vi "Test Assert Greater Or Equal.vi"(8 "error in (no error)":errorcluster) -> (0 "error out":errorcluster)   [LabVIEW 2020]
uses:
  classes/Assert/Assert.lvclass
  classes/Test/Test.lvclass
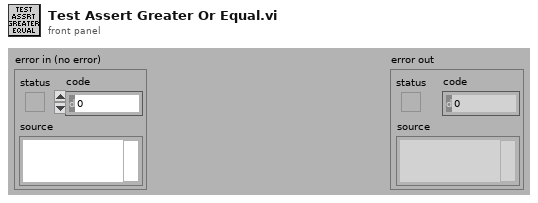
[diagram p1: front panel]
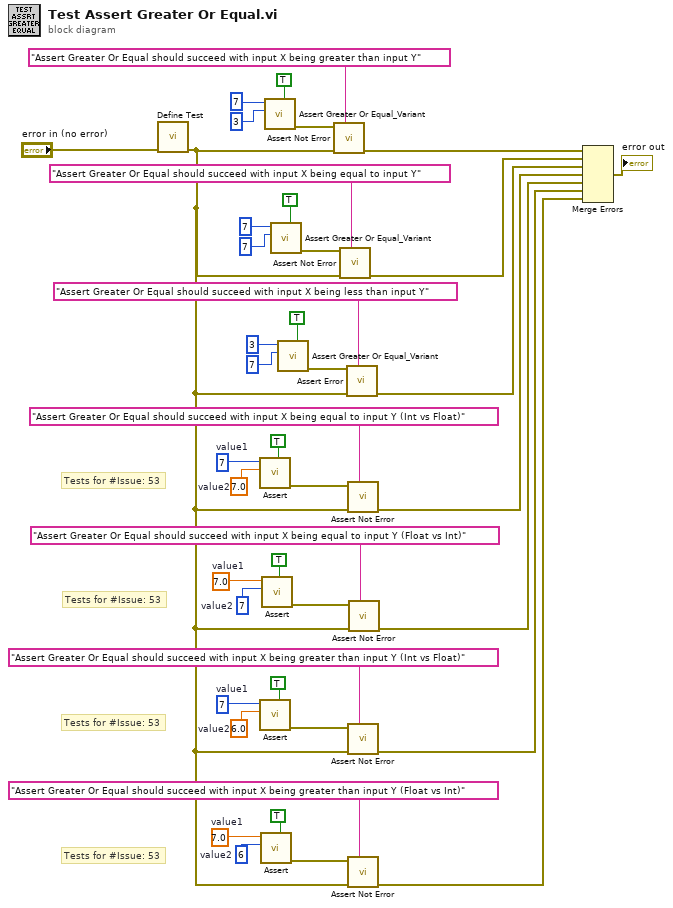
[diagram p0: block diagram]
diagram:
  w14 = 6  # value2
  w15 = 7.0  # value1
  w5 = 7  # value2
  w6 = 7.0  # value1
  w10 = 6.0  # value2
  w11 = 7  # value1
  w2 = 7.0  # value2
  w3 = 7  # value1
  # "Tests for #Issue: 53"
  # "Tests for #Issue: 53"
  # "Tests for #Issue: 53"
  # "Tests for #Issue: 53"
  n1 = call "Define Test.vi"("error in (no error)"="error in (no error)") -> ("error out"=w18:errorcluster)  [unwired: 9 in, 1 out]
  n2 = call-poly "Assert.vi"("Assert Only? (F)"=TRUE, "Y"=w2, "X"=w3) -> ("error out"=w1:errorcluster)  [unwired: 7 in, 1 out]
  n3 = call-poly "Assert.vi"("Assert Only? (F)"=TRUE, "Y"=w10, "X"=w11) -> ("error out"=w12:errorcluster)  [unwired: 7 in, 1 out]
  n4 = call-poly "Assert.vi"("Assert Only? (F)"=TRUE, "Y"=w14, "X"=w15) -> ("error out"=w13:errorcluster)  [unwired: 7 in, 1 out]
  n5 = call-poly "Assert.vi"("Assert Only? (F)"=TRUE, "Y"=w5, "X"=w6) -> ("error out"=w7:errorcluster)  [unwired: 7 in, 1 out]
  n6 = call "Assert Greater Or Equal_Variant.vi"("Assert Only? (F)"=TRUE, "Y"=3, "X"=7) -> ("error out"=w45:errorcluster)  [unwired: 7 in, 1 out]
  n7 = call "Assert Greater Or Equal_Variant.vi"("Assert Only? (F)"=TRUE, "Y"=7, "X"=7) -> ("error out"=w43:errorcluster)  [unwired: 7 in, 1 out]
  n8 = call "Assert Greater Or Equal_Variant.vi"("Assert Only? (F)"=TRUE, "Y"=7, "X"=3) -> ("error out"=w31:errorcluster)  [unwired: 7 in, 1 out]
  n9 = call "Assert Not Error.vi"("Label"="Assert Greater Or Equal should succeed with input X being greater than input Y", "error in (no error)"=w18, "Not Error?"=w45) -> ("error out"=w37:errorcluster)  [unwired: 7 in, 1 out]
  n10 = call "Assert Not Error.vi"("Label"="Assert Greater Or Equal should succeed with input X being equal to input Y", "error in (no error)"=w18, "Not Error?"=w43) -> ("error out"=w38:errorcluster)  [unwired: 7 in, 1 out]
  n11 = call "Assert Error.vi"("Label"="Assert Greater Or Equal should succeed with input X being less than input Y", "error in (no error)"=w18, "Error?"=w31) -> ("error out"=w26:errorcluster)  [unwired: 7 in, 1 out]
  n12 = call "Assert Not Error.vi"("Label"="Assert Greater Or Equal should succeed with input X being equal to input Y (Int vs Float)", "error in (no error)"=w18, "Not Error?"=w1) -> ("error out"=w25:errorcluster)  [unwired: 7 in, 1 out]
  n13 = call "Assert Not Error.vi"("Label"="Assert Greater Or Equal should succeed with input X being greater than input Y (Int vs Float)", "error in (no error)"=w18, "Not Error?"=w12) -> ("error out"=w22:errorcluster)  [unwired: 7 in, 1 out]
  n14 = call "Assert Not Error.vi"("Label"="Assert Greater Or Equal should succeed with input X being greater than input Y (Float vs Int)", "error in (no error)"=w18, "Not Error?"=w13) -> ("error out"=w17:errorcluster)  [unwired: 7 in, 1 out]
  n15 = call "Assert Not Error.vi"("Label"="Assert Greater Or Equal should succeed with input X being equal to input Y (Float vs Int)", "error in (no error)"=w18, "Not Error?"=w7) -> ("error out"=w20:errorcluster)  [unwired: 7 in, 1 out]
  n16 = Merge Errors(w37, w38, w26, w25, w20, w22, w17) -> (→"error out":errorcluster)
